vi "Generate Single Overlay.vi"(6 "Temp In":T1, 8 "error in":errorcluster, 9 "Single Color":bool, 10 "Overlay":T2, 11 "BigMAQ in":refnum<class "BigMAQ.lvclass">) -> (0 "error out":errorcluster, 2 "Overlay Out":T2, 3 "BigMAQ out":refnum<class "BigMAQ.lvclass">, 4 "Temp Out":T1)   [LabVIEW 2019, in "BigMAQ.lvclass"]
uses:
  BigMAQ.lvclass
  Overlay.ctl
  <vilib>/vision/Image Controls.llb/IMAQ Image.ctl
  BigMAQ.lvclass/BigMAQ.ctl
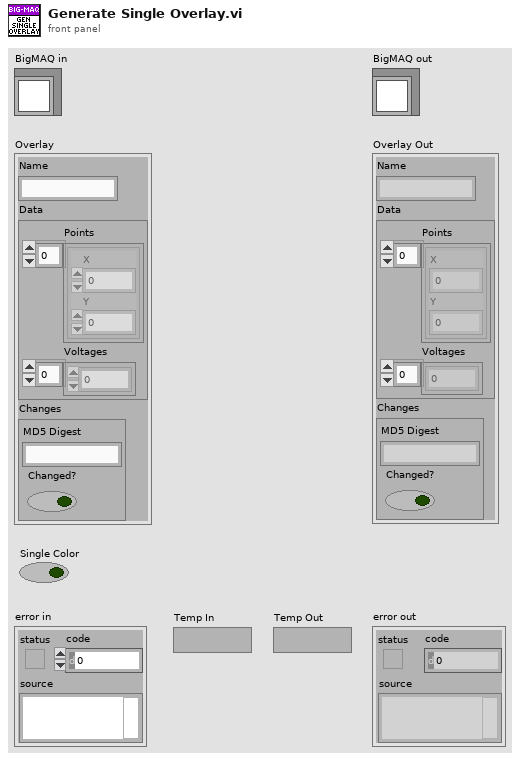
[diagram p1: front panel]
types:
  T1 = typedef "IMAQ Image.ctl" = refnum<image>
  T2 = typedef "BigMAQ.lvclass/Overlay.ctl" = cluster{"Name":string, "Data":cluster{"Points":cluster{"X":dbl, "Y":dbl}[], "Voltages":dbl[]}, "Changes":cluster{"MD5 Digest":string, "Changed?":bool}}
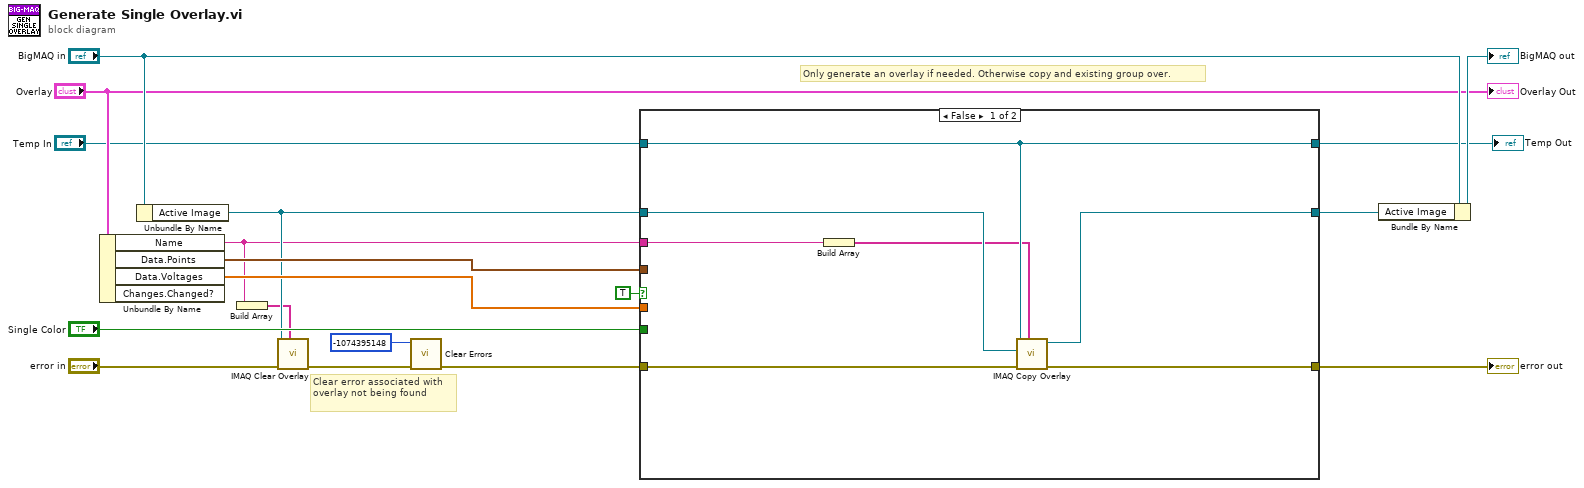
[diagram p0: block diagram]
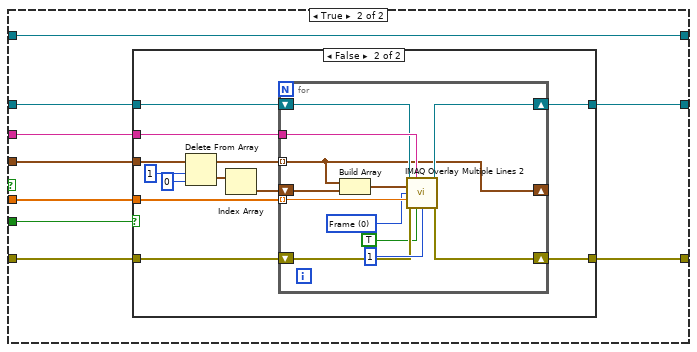
[diagram p2: hidden frame]
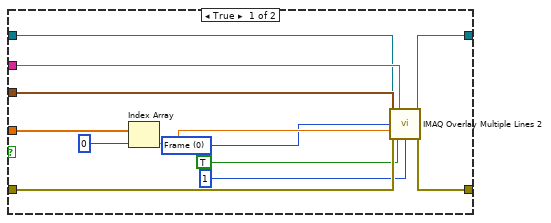
[diagram p3: hidden frame]
diagram:
  # "Only generate an overlay if needed. Otherwise copy and existing group over."
  # "Clear error associated with overlay not being found"
  n1 = Unbundle By Name("Overlay") -> ("Name"=w2:string, "Data.Points"=w18:cluster{"X":dbl, "Y":dbl}[], "Data.Voltages"=w17:dbl[])  [unwired: 1 out]
  n2 = Unbundle By Name("BigMAQ in") -> ("Active Image"=w3:T1)
  n3 = Build Array(w2) -> (w1:string[])
  n4 = call "IMAQ Clear Overlay"("Groups"=w1, "error in (no error)"="error in", "Image"=w3) -> ("error out"=w4:errorcluster)  [unwired: 7 in, 1 out]
  n5 = call <vilib>:"Clear Errors.vi"("error in (no error)"=w4, "specific error code to clear (0: all)"=-1074395148) -> ("error out"=w10:errorcluster)  [unwired: 4 in, 1 out]
  n6 = case shown="False" TRUE {
    tunnel: w18 -> [_ w34]
    tunnel: w17 -> [_ w33]
    tunnel: [w24 w32] -> w16
    tunnel: "Single Color" -> [_ w31]
    tunnel: [w22 w30] -> w11
    tunnel: w2 -> [w20 w29]
    tunnel: w10 -> [w21 w28]
    tunnel: w3 -> [w23 w27]
    tunnel: "Temp In" -> [w25 w26]
    tunnel: [w25 w26] -> w7
    frame False {
      n7 = Build Array(w20) -> (w19:string[])
      n8 = call "IMAQ Copy Overlay"("Groups"=w19, "error in (no error)"=w21, "Image Dst"=w23, "Image Src"=w25) -> ("error out"=w22:errorcluster, "Image Dst Out"=w24:T1)  [unwired: 6 in]
    }
    frame True {
      n9 = case shown="False" w31 {
        tunnel: w27 -> [w38 w58]
        tunnel: w29 -> [w46 w57]
        tunnel: w28 -> [w45 w56]
        tunnel: [w39 w55] -> w30
        tunnel: w34 -> [w44 w49]
        tunnel: [w42 w54] -> w32
        tunnel: w33 -> [w41 w53]
        frame True {
          w36 = u32 0 items=["Frame", "Fill"] ("Drawing Mode (Frame)")
          n10 = Index Array(array=w41, index=0) -> (element=w40:dbl)
          n11 = call "IMAQ Overlay Multiple Lines 2"("Image"=w38, "Group"=w46, "Line End Points"=w44, "Drawing Mode (Frame)"=w36, "Color"=w40, "error in (no error)"=w45, "Maintain Width?"=TRUE, "Width"=u32 1) -> ("Image Out"=w42:T1, "error out"=w39:errorcluster)  [unwired: 6 in]
        }
        frame False {
          n12 = Delete From Array(array=w49, length=1, index=0) -> (deleted portion=w48:cluster{"X":dbl, "Y":dbl}[], array with subset deleted=w50:cluster{"X":dbl, "Y":dbl}[])
          n13 = Index Array(array=w48) -> (element=w47:cluster{"X":dbl, "Y":dbl})  [unwired: 1 in]
          n14 = for {
            tunnel: w57 -> [w70]
            tunnel: w50 -> [w60] mode=indexing
            shift-right: [w68] -> w54
            shift-left: w58 -> [w67]
            shift-right: [w66] -> w55
            shift-left: w56 -> [w65]
            tunnel: w53 -> [w63] mode=indexing
            shift-right: [w60] -> _
            shift-left: w47 -> [w61]
            w62 = u32 0 items=["Frame", "Fill"] ("Drawing Mode (Frame)")
            n15 = Build Array(w60, w61) -> (w59:cluster{"X":dbl, "Y":dbl}[])
            n16 = call "IMAQ Overlay Multiple Lines 2"("Image"=w67, "Group"=w70, "Line End Points"=w59, "Drawing Mode (Frame)"=w62, "Color"=w63, "error in (no error)"=w65, "Maintain Width?"=TRUE, "Width"=u32 1) -> ("Image Out"=w68:T1, "error out"=w66:errorcluster)  [unwired: 6 in]
          }
        }
      }
    }
  }
  "error out" <- w11
  "Temp Out" <- w7
  n17 = Bundle By Name(cluster="BigMAQ in", "Active Image"=w16) -> (→"BigMAQ out":refnum<class "BigMAQ.lvclass">)
  "Overlay Out" <- "Overlay"
